vi "waveform control.vi"() -> ()   [LabVIEW 2018]
panel:
  out "Waveform Graph 2":dbl[](graph)
  in  "length 2":dbl
  in  "index":dbl
  in  "Amplitude":dbl(knob) scale=0.0..10.0
  in  "Frequency":dbl
  in  "stop":bool
  out "Waveform Graph":dynamicdata(graph)
  # "Waveform control"
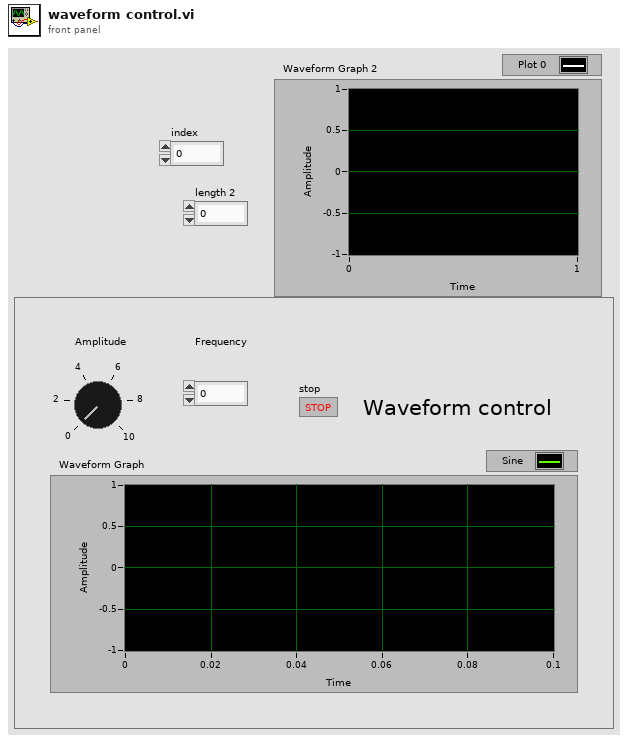
[diagram p1: front panel]
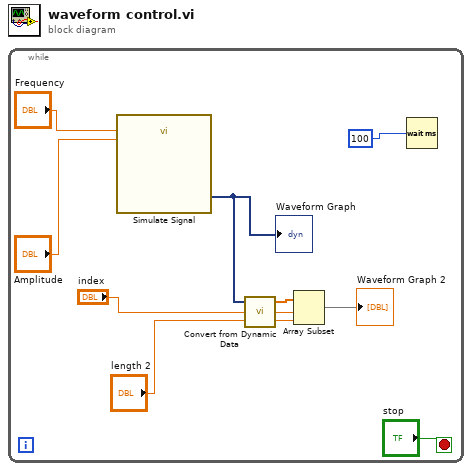
[diagram p0: block diagram]
diagram:
  n1 = while {
    stop <- "stop" stop-if-true
    n2 = call "Simulate Signal"("Frequency"="Frequency", "Amplitude"="Amplitude") -> ("Sine"=w5:dynamicdata)  [unwired: 12 in, 1 out]
    "Waveform Graph" <- w5
    n3 = call "Convert from Dynamic Data"("Dynamic Data Type"=w5) -> ("Array"=w4:dbl[])  [unwired: 3 in]
    n4 = Array Subset "Array Subset"(array=w4, index="index", length="length 2") -> (→"Waveform Graph 2":dbl[])
    n5 = Wait (ms)(milliseconds to wait=100) -> ()  [unwired: 1 out]
  }
